vi "Client Single Connection.vi"() -> ()   [LabVIEW 2013]
doc: "This WebSockets API example VI acts as a client to make an outgoing websockets connection. Receives/sends string data to the connected server."
uses:
  WebSockets/WebSocket Client/WebSocket Client.lvclass
  WebSockets/WebSocket/WebSocket.lvclass/WebSocket.ctl
  WebSockets/WebSocket/WebSocket.lvclass
panel:
  in  "Disconnect":bool
  in  "Connect":bool
  in  "WebSockets URL":string="ws://echo.websocket.org"
  out "HTTP Headers":variant
  in  "Stop":bool
  out "Received Data":string
  in  "Send":bool
  in  "Data":string
  # "WebSockets Client Example"
  # "This VI is a simple example of sending/receiving data using WebSockets.\nIt opens a WebSockets Client connection to the WebSockets URL and can send / receive WebSockets data from the server.\n\nInstructions for use:\n1) Run this VI\n2) Enter the WebSockets URL that you wish to open a connection to (e.g. ws://echo.websocket.org) and click 'Connect'\n3) Enter text to send in 'Data' hit 'Send' to send to the WebSockets server\n4) WebSockets messages received from the server will be displayed in 'Received Data'"
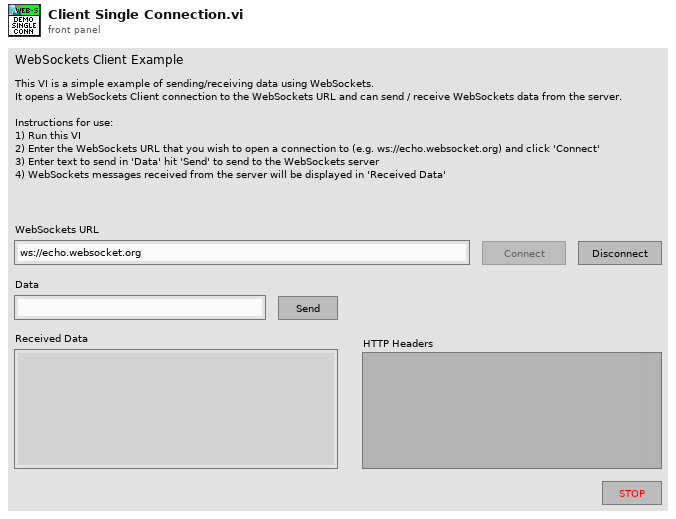
[diagram p1: front panel]
types:
  T1 = enum8{"Enabled", "Disabled", "Disabled and Grayed Out"}
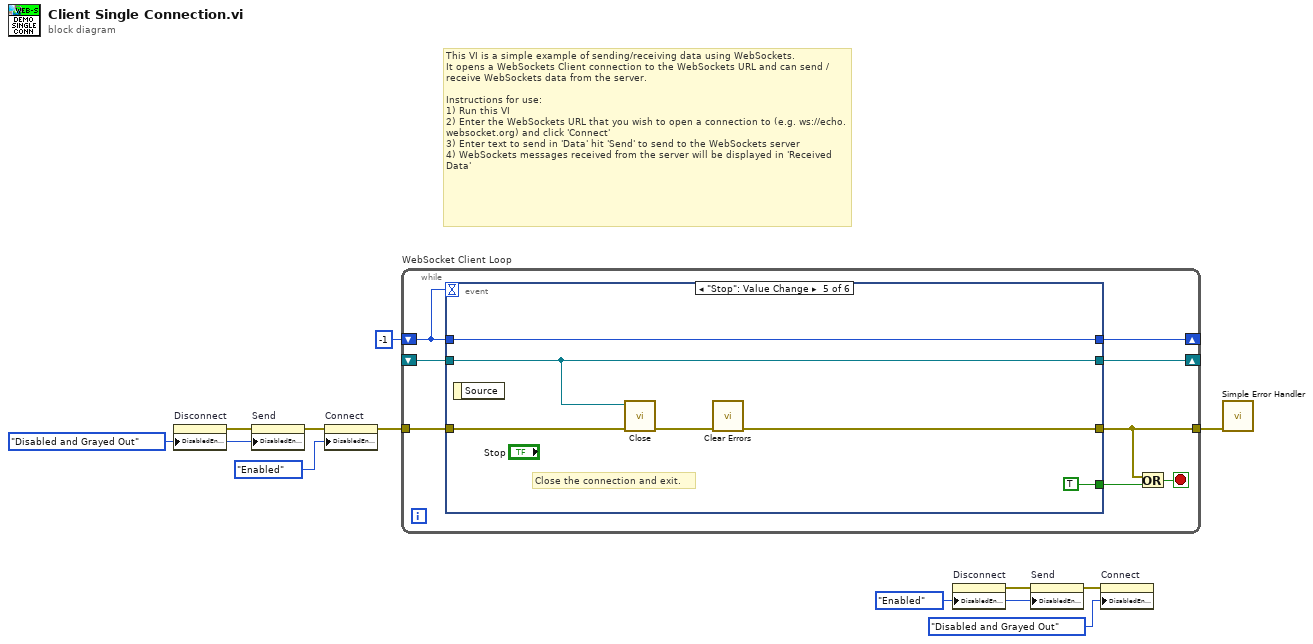
[diagram p0: block diagram]
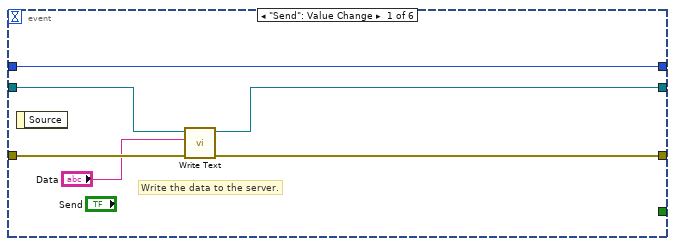
[diagram p2: hidden frame]
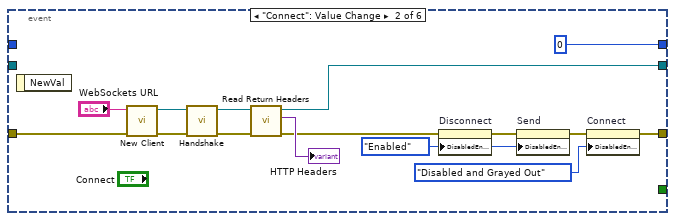
[diagram p3: hidden frame]
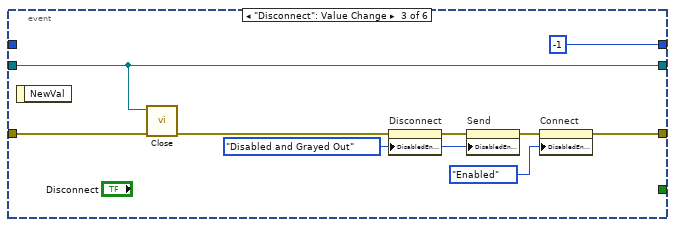
[diagram p4: hidden frame]
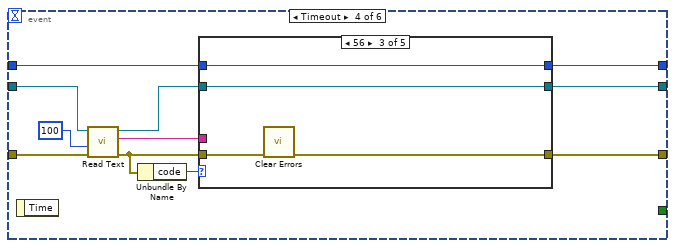
[diagram p5: hidden frame]
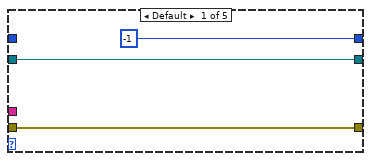
[diagram p6: hidden frame]
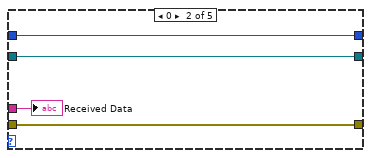
[diagram p7: hidden frame]
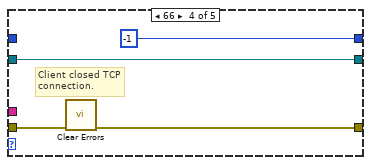
[diagram p8: hidden frame]
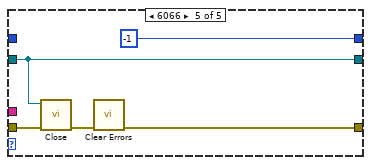
[diagram p9: hidden frame]
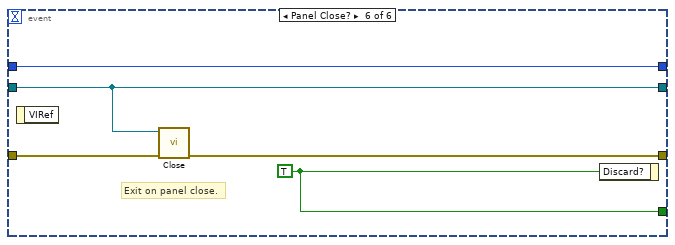
[diagram p10: hidden frame]
diagram:
  w4 = T1."Enabled" ("Disabled")
  w8 = T1."Disabled and Grayed Out" ("Disabled")
  # "This VI is a simple example of sending/receiving data using WebSockets.\nIt opens a WebSockets Client connection to the WebSockets URL and can send / receive WebSockets data from the server.\n\nInstructions for use:\n1) Run this VI\n2) Enter the WebSockets URL that you wish to open a connection to (e.g. ws://echo.websocket.org) and click 'Connect'\n3) Enter text to send in 'Data' hit 'Send' to send to the WebSockets server\n4) WebSockets messages received from the server will be displayed in 'Received Data'"
  n1 = property on="Disconnect" class="Bool"("DisabledEnum"=w8) -> (error out=w9:errorcluster)  [unwired: 2 in, 1 out]
  n2 = property on="Send" class="Bool"(error in=w9, "DisabledEnum"=w8) -> (error out=w3:errorcluster)  [unwired: 1 in, 1 out]
  n3 = property on="Connect" class="Bool"(error in=w3, "DisabledEnum"=T1."Enabled" ("Disabled")) -> (error out=w2:errorcluster)  [unwired: 1 in, 1 out]
  n4 = while "WebSocket Client Loop" {
    tunnel: [w16] -> w11
    tunnel: w2 -> [w19]
    shift-right: [w15] -> _
    shift-left: _ -> [w14]
    shift-right: [w13] -> _
    shift-left: -1 -> [w12]
    stop <- w17 stop-if-true
    n5 = event shown="[4] \"Stop\": Value Change" {
      selector: _ -> [_ _ _ _ _ _]
      dyn-events: _ -> [_ _ _ _ _ _]
      timeout: w12 -> [_ _ _ _ _ _]
      tunnel: [_ _ _ _ TRUE w91] -> w18
      tunnel: [w24 w27 w41 w55 w81 w89] -> w16
      tunnel: w19 -> [w25 w39 w49 w60 w85 w90]
      tunnel: [w21 w34 w48 w52 w83 w88] -> w15
      tunnel: w14 -> [w22 _ w48 w59 w83 w88]
      tunnel: w12 -> [w20 _ _ w51 w82 w87]
      tunnel: [w20 0 -1 w50 w82 w87] -> w13
      event "Send": Value Change {
        # "Write the data to the server."
        n6 = event-data() -> ()  [unwired: 1 in, 1 out]
        n7 = call-dynamic "Write Text.vi"("error in (no error)"=w25, "String Data"="Data", "WebSocket in"=w22) -> ("error out"=w24:errorcluster, "WebSocket out"=w21:refnum<class "WebSocket Client.lvclass">)  [unwired: 7 in]
      }
      event "Connect": Value Change {
        w31 = T1."Enabled" ("Disabled")
        n8 = event-data() -> ()  [unwired: 1 in, 1 out]
        n9 = call "New Client.vi"("error in (no error)"=w39, "WebSocket URL"="WebSockets URL") -> ("error out"=w40:errorcluster, "WebSocket Client out"=w37:refnum<class "WebSocket Client.lvclass">)  [unwired: 8 in]
        n10 = call-dynamic "Handshake.vi"("error in (no error)"=w40, "WebSocket Client in"=w37) -> ("error out"=w36:errorcluster, "WebSocket Client out"=w35:refnum<class "WebSocket Client.lvclass">)  [unwired: 8 in]
        n11 = call "Read Return Headers.vi"("error in (no error)"=w36, "WebSocket in"=w35) -> ("error out"=w29:errorcluster, "Return Headers"=→"HTTP Headers":variant, "WebSocket out"=w34:refnum<class "WebSocket Client.lvclass">)  [unwired: 7 in]
        n12 = property on="Disconnect" class="Bool"(error in=w29, "DisabledEnum"=w31) -> (error out=w30:errorcluster)  [unwired: 1 in, 1 out]
        n13 = property on="Send" class="Bool"(error in=w30, "DisabledEnum"=w31) -> (error out=w28:errorcluster)  [unwired: 1 in, 1 out]
        n14 = property on="Connect" class="Bool"(error in=w28, "DisabledEnum"=T1."Disabled and Grayed Out" ("Disabled")) -> (error out=w27:errorcluster)  [unwired: 1 in, 1 out]
      }
      event "Disconnect": Value Change {
        w44 = T1."Disabled and Grayed Out" ("Disabled")
        n15 = event-data() -> ()  [unwired: 1 in, 1 out]
        n16 = call-dynamic "Close.vi"("error in (no error)"=w49, "WebSocket in"=w48) -> ("error out"=w42:errorcluster)  [unwired: 9 in]
        n17 = property on="Disconnect" class="Bool"(error in=w42, "DisabledEnum"=w44) -> (error out=w43:errorcluster)  [unwired: 1 in, 1 out]
        n18 = property on="Send" class="Bool"(error in=w43, "DisabledEnum"=w44) -> (error out=w45:errorcluster)  [unwired: 1 in, 1 out]
        n19 = property on="Connect" class="Bool"(error in=w45, "DisabledEnum"=T1."Enabled" ("Disabled")) -> (error out=w41:errorcluster)  [unwired: 1 in, 1 out]
      }
      event Timeout {
        n20 = event-data() -> ()  [unwired: 1 in, 1 out]
        n21 = call-dynamic "Read Text.vi"("error in (no error)"=w60, "timeout ms (5000)"=100, "WebSocket in"=w59) -> ("error out"=w54:errorcluster, "Data"=w57:string, "WebSocket out"=w53:refnum<class "WebSocket Client.lvclass">)  [unwired: 6 in]
        n22 = Unbundle By Name(w54) -> ("code"=w56:i32)
        n23 = case shown="56" w56 {
          tunnel: w57 -> [_ w67 _ _ _]
          tunnel: [w63 w66 w70 w72 w76] -> w55
          tunnel: w54 -> [w63 w66 w71 w75 w80]
          tunnel: w53 -> [w62 w65 w69 w74 w78]
          tunnel: [w62 w65 w69 w74 w78] -> w52
          tunnel: w51 -> [_ w64 w68 _ _]
          tunnel: [-1 w64 w68 -1 -1] -> w50
          frame Default {
          }
          frame 0 {
            "Received Data" <- w67
          }
          frame 56 {
            n24 = call <vilib>:"Clear Errors.vi"("error in (no error)"=w71) -> ("error out"=w70:errorcluster)  [unwired: 6 in]
          }
          frame 66 {
            # "Client closed TCP connection."
            n25 = call <vilib>:"Clear Errors.vi"("error in (no error)"=w75) -> ("error out"=w72:errorcluster)  [unwired: 6 in]
          }
          frame 6066 {
            n26 = call-dynamic "Close.vi"("error in (no error)"=w80, "WebSocket in"=w78) -> ("error out"=w79:errorcluster)  [unwired: 9 in]
            n27 = call <vilib>:"Clear Errors.vi"("error in (no error)"=w79) -> ("error out"=w76:errorcluster)  [unwired: 6 in]
          }
        }
      }
      event "Stop": Value Change {
        # "Close the connection and exit."
        n28 = event-data() -> ()  [unwired: 1 in, 1 out]
        n29 = call-dynamic "Close.vi"("error in (no error)"=w85, "WebSocket in"=w83) -> ("error out"=w84:errorcluster)  [unwired: 9 in]
        n30 = call <vilib>:"Clear Errors.vi"("error in (no error)"=w84) -> ("error out"=w81:errorcluster)  [unwired: 6 in]
      }
      event Panel Close? {
        w91 = TRUE ("Discard?")
        # "Exit on panel close."
        n31 = event-data() -> ()  [unwired: 1 in, 1 out]
        n32 = call-dynamic "Close.vi"("error in (no error)"=w90, "WebSocket in"=w88) -> ("error out"=w89:errorcluster)  [unwired: 9 in]
        n33 = event-data("Discard?"=w91) -> ()  [unwired: 1 in, 1 out]
      }
    }
    n34 = Or(x=w16, y=w18) -> (x .or. y?=w17:bool)
  }
  n35 = property on="Disconnect" class="Bool"("DisabledEnum"=w4) -> (error out=w5:errorcluster)  [unwired: 2 in, 1 out]
  n36 = property on="Send" class="Bool"(error in=w5, "DisabledEnum"=w4) -> (error out=w6:errorcluster)  [unwired: 1 in, 1 out]
  n37 = property on="Connect" class="Bool"(error in=w6, "DisabledEnum"=T1."Disabled and Grayed Out" ("Disabled")) -> ()  [unwired: 1 in, 2 out]
  n38 = call <vilib>:"Simple Error Handler.vi"("error in (no error)"=w11) -> ()  [unwired: 4 in, 5 out]
